vi "user32 SetKeyboardState.vi"(0 "key state":u8[](array[numeric]), 11 "error in":errorcluster) -> (4 "return value":i32, 15 "error out":errorcluster)   [LabVIEW 2020, in "RemoteVI.lvlib"]
doc: "Replaces the key state of the CALLING thread through user32.dll SetKeyboardState (stdcall, called in LabVIEW's UI thread). Only that thread's state changes - not the physical keyboard, not GetAsyncKeyState, not any other program. Running in the UI thread, this sets what LabVIEW's panels read for the modifier keys, until the thread next retrieves real input from the host's keyboard or mouse. key state is cut or padded with zeros to the 256 bytes the function reads. return value is the Win32 BOOL: non-zero on success, 0 on failure. When error in carries an error the DLL is not called. Generated by scripts\\Build Win32 Wrappers.vi - do not edit by hand, rebuild it."
uses:
  RemoteVI.lvlib
  user32.dll
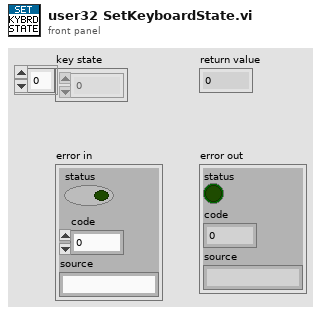
[diagram p1: front panel]
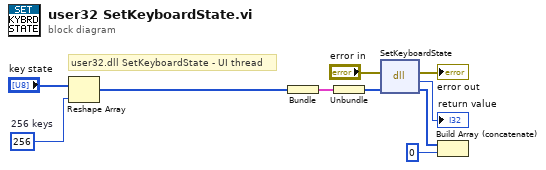
[diagram p0: block diagram]
diagram:
  w8 = 256  # 256 keys
  # "user32.dll SetKeyboardState - UI thread"
  n1 = Reshape Array("key state", w8) -> (w9:u8[])
  n2 = Bundle("key state"=w9) -> (w10:cluster{"key state":u8[]})  [unwired: 1 in]
  n3 = Unbundle(w10) -> ("key state"=w2:u8[])
  n4 = dll-call lib="user32.dll" fn="SetKeyboardState"(error in="error in", "lpKeyState"=w2) -> (error out=→"error out":errorcluster, →"return value":i32, "lpKeyState"=w1:u8[])  [unwired: 2 in, 1 out]
  n5 = Build Array (concatenate)(w1, u8 0) -> ()  [unwired: 1 out]
